vi "Write Scalar Data.vi"(8 "error in (no error)":errorcluster, 9 "Changed?":bool[](array[boolean]), 10 "Values":dbl[](array[numeric]), 11 "Cluster":T1 {"Data Type" format="%.0x"}) -> (0 "error out":errorcluster, 2 "Values":dbl[](array[numeric]), 3 "Cluster":T1 {"Data Type" format="%.0x"})   [LabVIEW 2019, in "FPGA Addon Engine.lvlib"]
uses:
  FPGA Addon Engine.lvlib
  Types/Register Settings.ctl
  Addon Shared/Types/Data Type.ctl
  Addon Shared/Types/Scalar Type.ctl
  <vilib>/Utility/error.llb/Error Cluster From Error Code.vi
  <vilib>/rvi/errors/niLvFpgaAdjustHostInterfaceError.vi
  <vilib>/rvi/interface/nirviReadWriteControl/nirviReadWriteControl.xnode
  <vilib>/rvi/interface/Simulation/niFpgaSimulationCallBeginRW.vi
  NiFpgaLv.dll
  Addon Shared/FPGA Addon Shared.lvlib
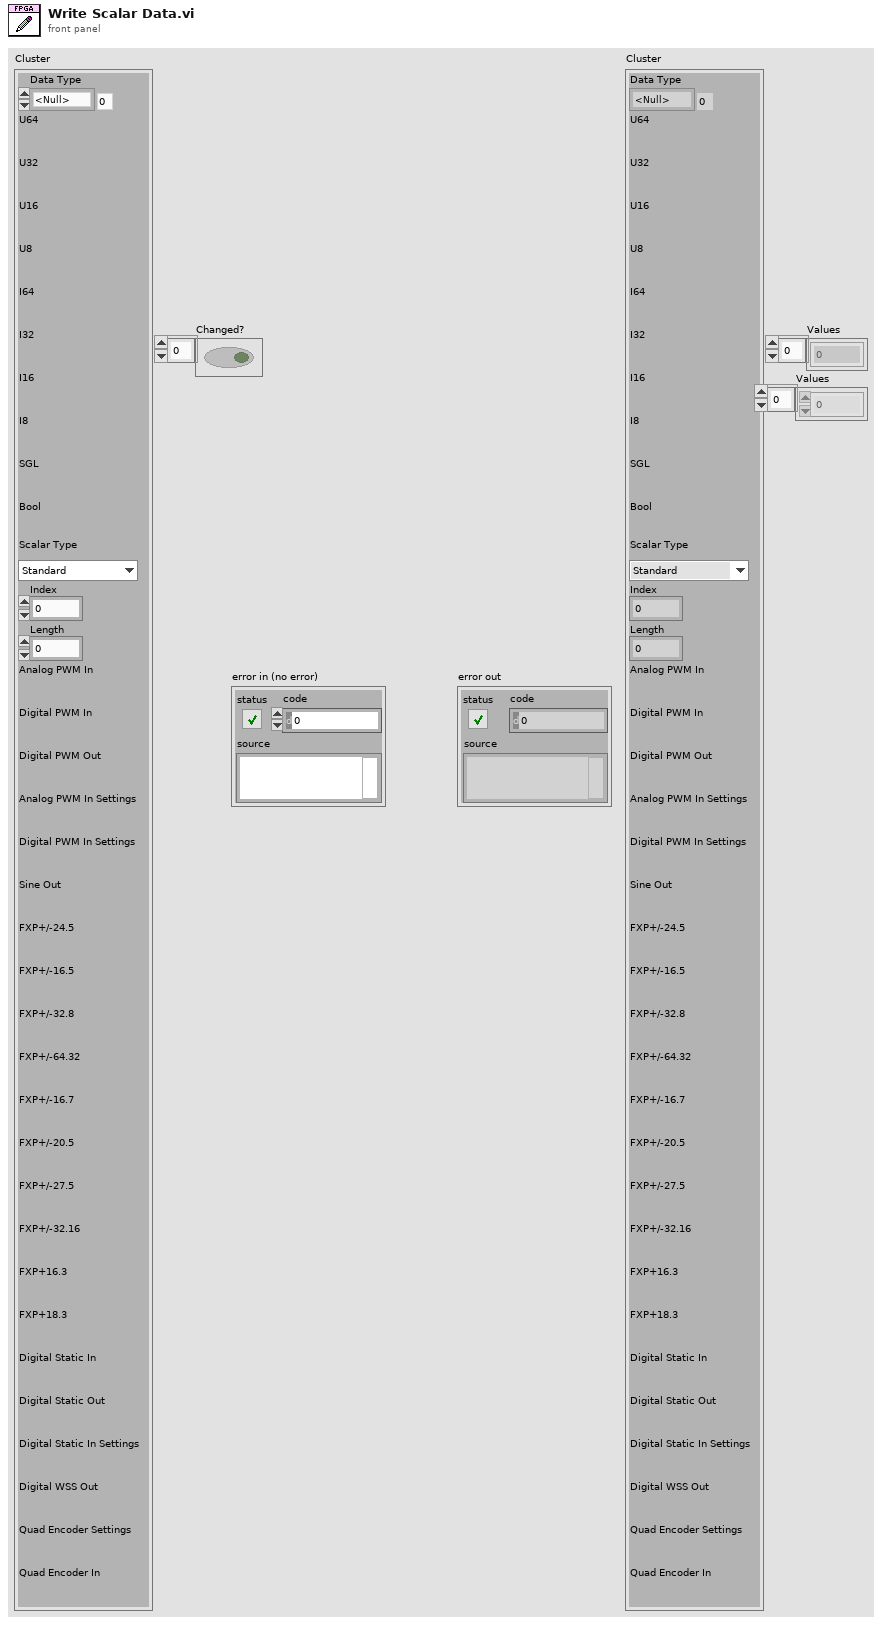
[diagram p1: front panel]
types:
  T1 = typedef "FPGA Addon Engine.lvlib/Register Settings.ctl" = cluster{"Data Type":T2, "U64":refnum<k20>, "U32":refnum<k20>, "U16":refnum<k20>, "U8":refnum<k20>, "I64":refnum<k20>, "I32":refnum<k20>, "I16":refnum<k20>, "I8":refnum<k20>, "SGL":refnum<k20>, "Bool":refnum<k20>, "Scalar Type":T3, "Index":i32, "Length":i32, "Analog PWM In":refnum<k20>, "Digital PWM In":refnum<k20>, "Digital PWM Out":refnum<k20>, "Analog PWM In Settings":refnum<k20>, "Digital PWM In Settings":refnum<k20>, "Sine Out":refnum<k20>, "FXP+/-24.5":refnum<k20>, "FXP+/-16.5":refnum<k20>, "FXP+/-32.8":refnum<k20>, "FXP+/-64.32":refnum<k20>, "FXP+/-16.7":refnum<k20>, "FXP+/-20.5":refnum<k20>, "FXP+/-27.5":refnum<k20>, "FXP+/-32.16":refnum<k20>, "FXP+16.3":refnum<k20>, "FXP+18.3":refnum<k20>, "Digital Static In":refnum<k20>, "Digital Static Out":refnum<k20>, "Digital Static In Settings":refnum<k20>, "Digital WSS Out":refnum<k20>, "Quad Encoder Settings":refnum<k20>, "Quad Encoder In":refnum<k20>}
  T2 = typedef "FPGA Addon Shared.lvlib/Data Type.ctl" = enum8{"<Null>", "I8", "I16", "I32", "I64", "U8", "U16", "U32", "U64", "SGL", "Boolean", "Analog PWM In Settings", "Analog PWM In", "Digital PWM In Settings", "Digital PWM In", "Digital PWM Out", "Sine Out", "FXP+/-24.5", "FXP+/-16.5", "FXP+/-32.8", "FXP+/-64.32", "FXP+/-16.7", "FXP+/-20.5", "FXP+/-27.5", "FXP+/-32.16", "FXP +16.3", "FXP +18.3", "Digital Static In", "Digital Static Out", "Digital Static In Settings", "Digital WSS Out", "Quad Encoder Settings", "Quad Encoder In"}
  T3 = typedef "FPGA Addon Shared.lvlib/Scalar Type.ctl" = enum16{"Standard", "Bitpacked"}
  T4 = cluster{"ACTIVE EDGE":bool, "TIMEOUT":u32, "THRESHOLD":fxp<+/-,32,8>}
  T5 = cluster{"ACTIVE EDGE":bool, "ACTIVE TICKS":u32, "INACTIVE TICKS":u32}
  T6 = cluster{"ACTIVE EDGE":bool, "ACTIVE TICKS":u32, "INACTIVE TICKS":u32, "DATA":u8, "SENSOR TYPE":u8}
  T7 = cluster{"AMP":fxp<+/-,32,8>, "OFFSET":fxp<+/-,32,8>, "PERIODS/TICKS":fxp<+,32,0>}
  T8 = cluster{"DIRECTION":u8, "RESET VALUE":i32, "A RESET STATE":bool, "B RESET STATE":bool, "Z RESET STATE":bool}
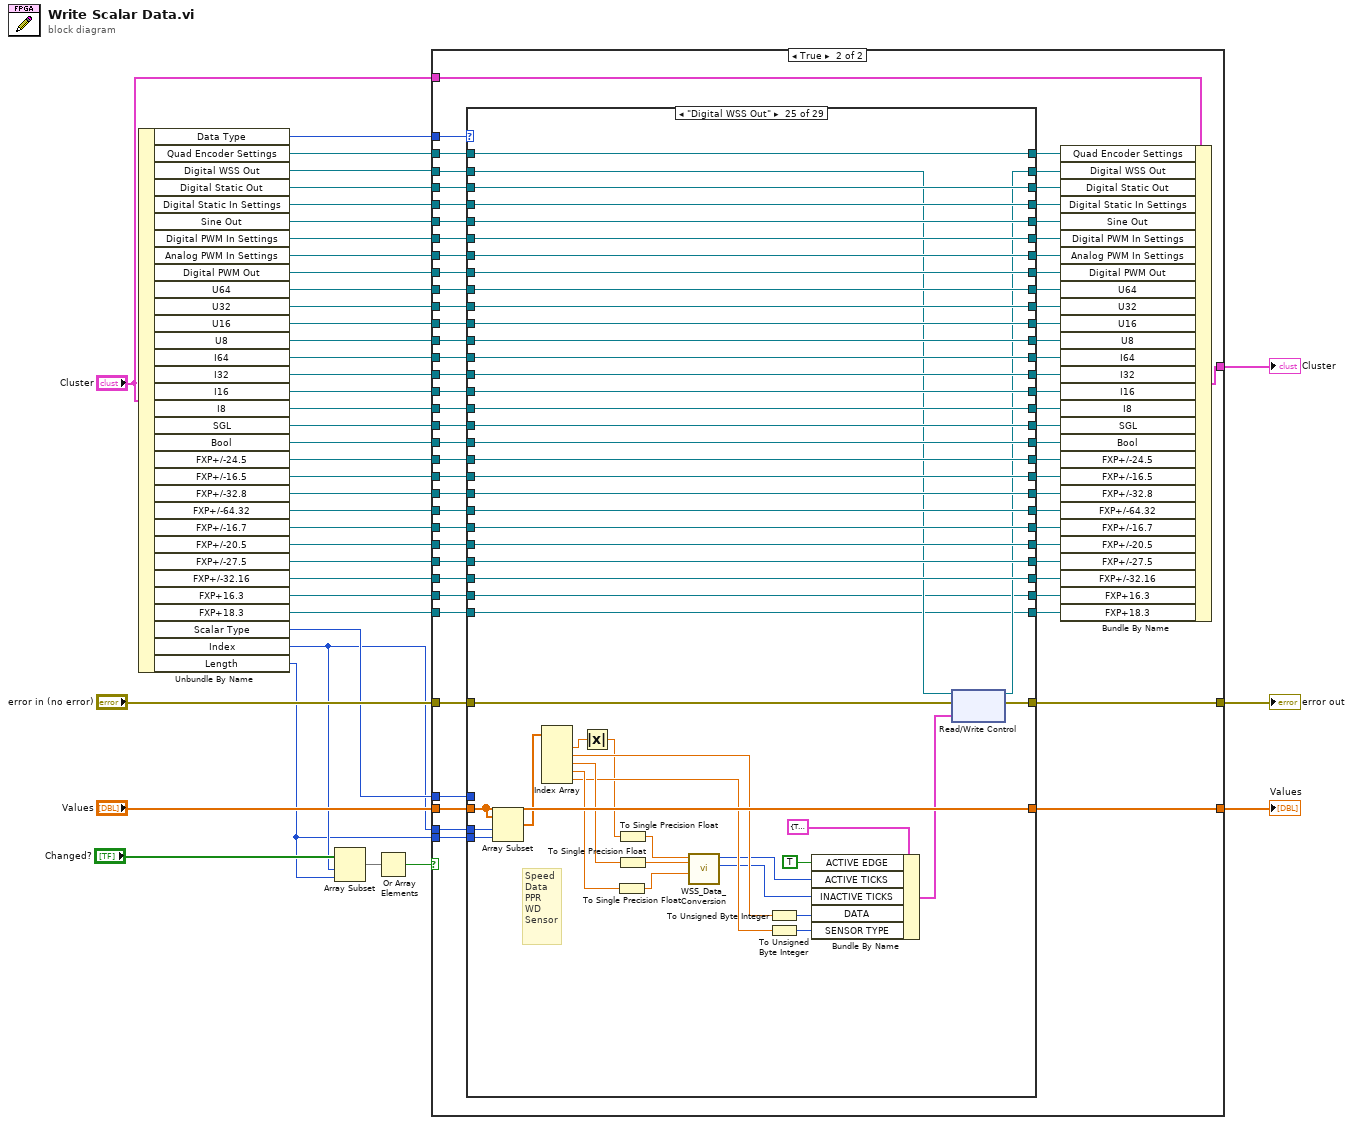
[diagram p0: block diagram]
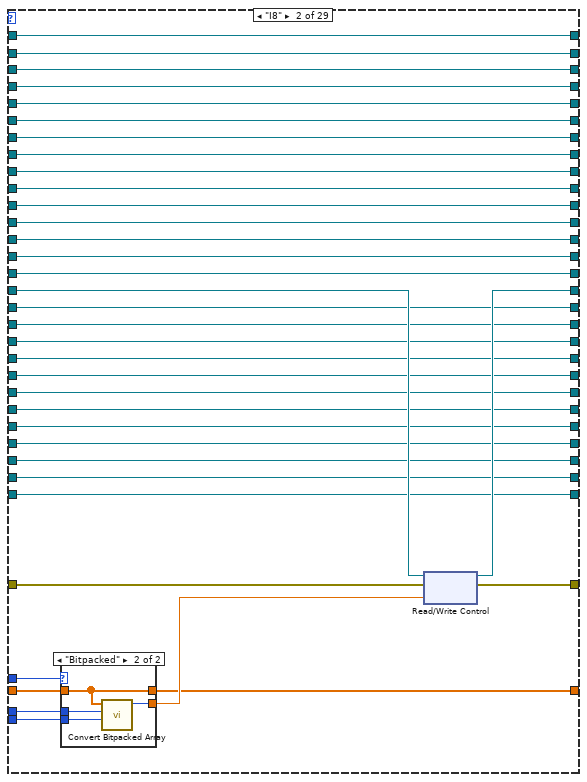
[diagram p4: hidden frame]
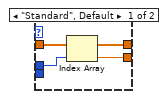
[diagram p5: hidden frame]
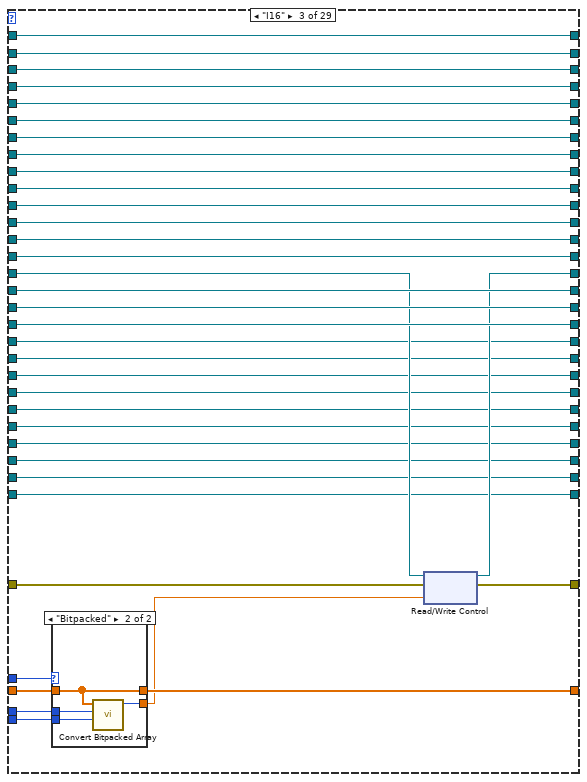
[diagram p6: hidden frame]
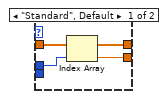
[diagram p7: hidden frame]
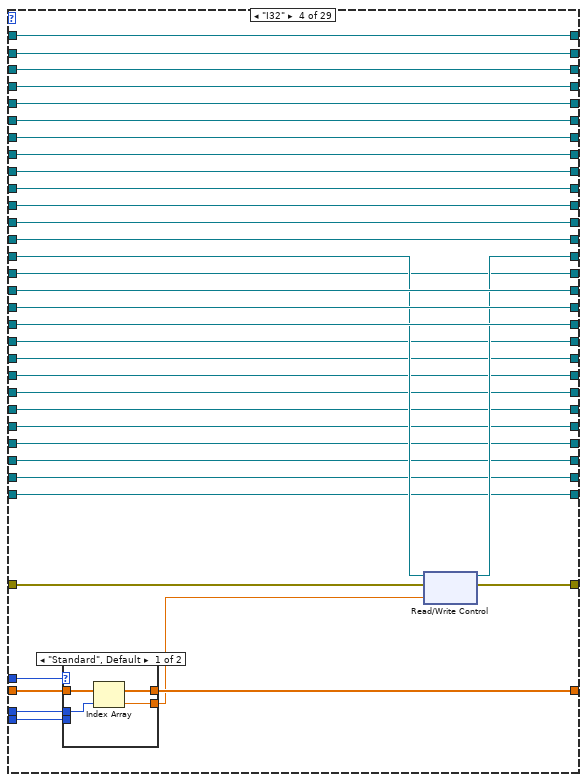
[diagram p8: hidden frame]
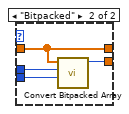
[diagram p9: hidden frame]
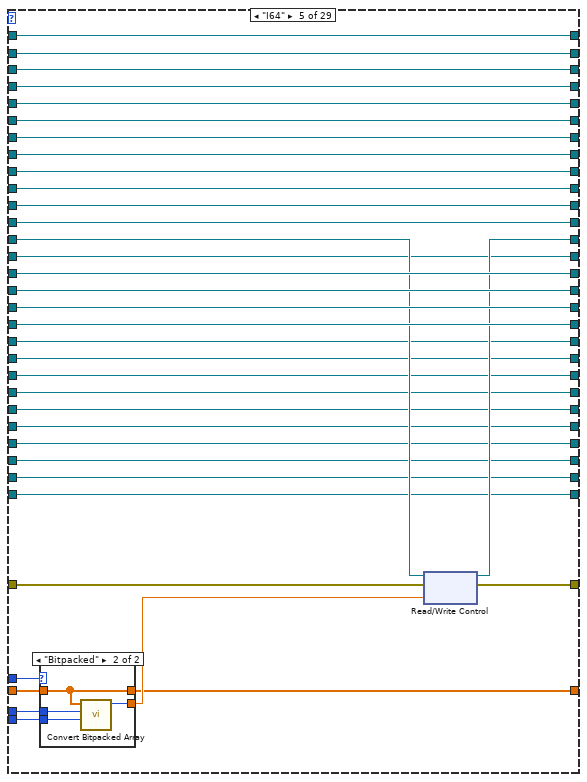
[diagram p10: hidden frame]
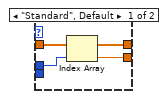
[diagram p11: hidden frame]
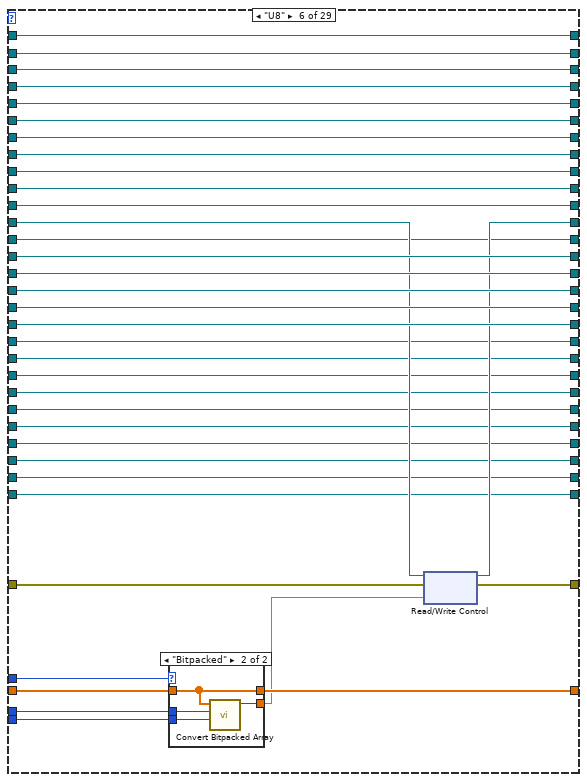
[diagram p12: hidden frame]
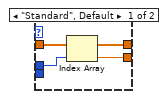
[diagram p13: hidden frame]
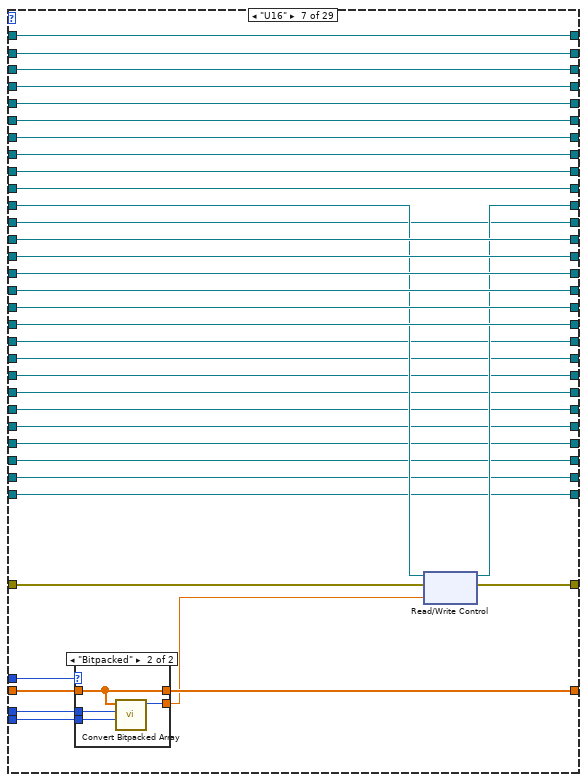
[diagram p14: hidden frame]
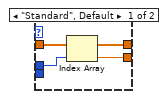
[diagram p15: hidden frame]
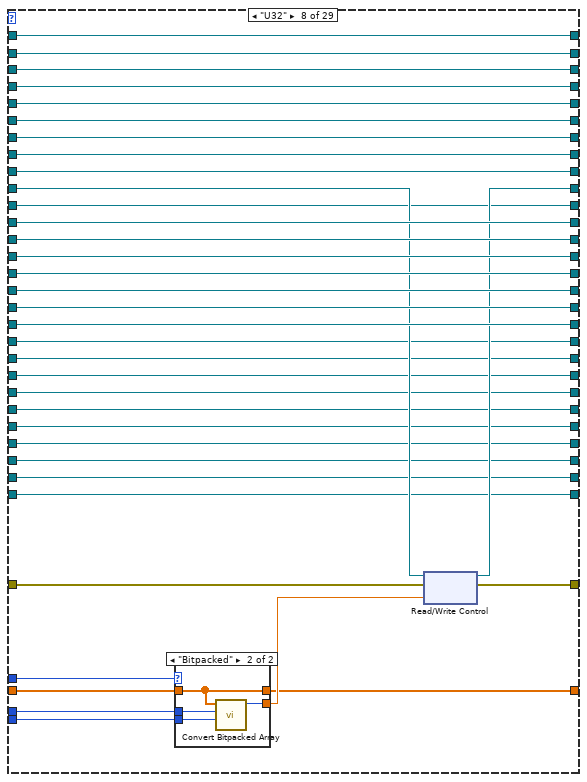
[diagram p16: hidden frame]
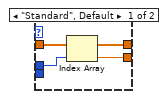
[diagram p17: hidden frame]
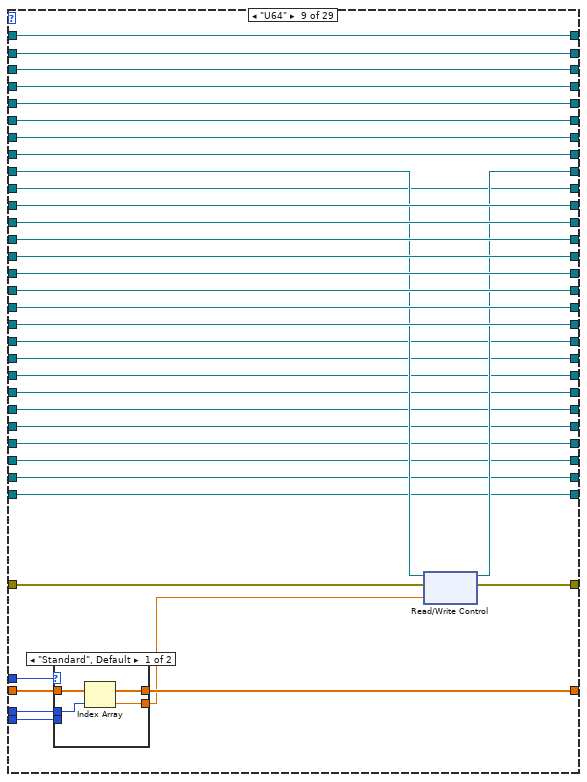
[diagram p18: hidden frame]
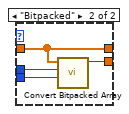
[diagram p19: hidden frame]
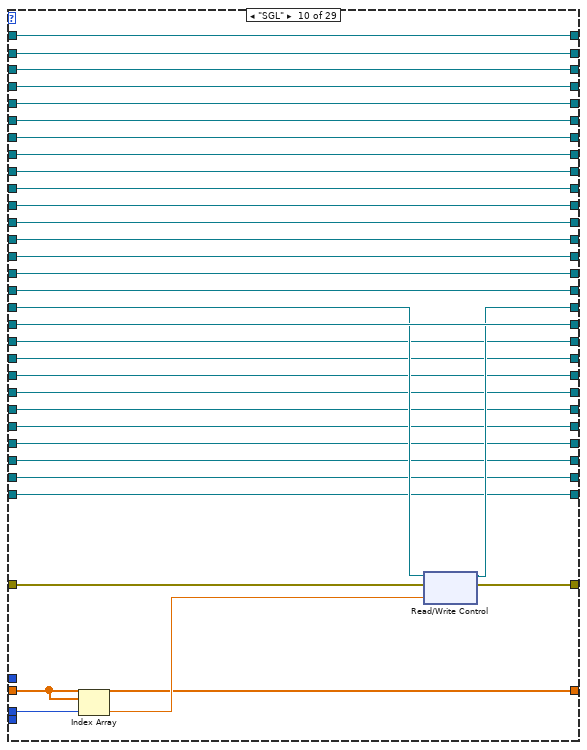
[diagram p20: hidden frame]
diagram:
  n1 = Unbundle By Name("Cluster") -> ("Data Type"=w4:T2, "Quad Encoder Settings"=w3:refnum<k20>, "Digital WSS Out"=w5:refnum<k20>, "Digital Static Out"=w7:refnum<k20>, "Digital Static In Settings"=w6:refnum<k20>, "Sine Out"=w16:refnum<k20>, "Digital PWM In Settings"=w22:refnum<k20>, "Analog PWM In Settings"=w23:refnum<k20>, "Digital PWM Out"=w24:refnum<k20>, "U64"=w29:refnum<k20>, "U32"=w30:refnum<k20>, "U16"=w31:refnum<k20>, "U8"=w32:refnum<k20>, "I64"=w33:refnum<k20>, "I32"=w34:refnum<k20>, "I16"=w35:refnum<k20>, "I8"=w41:refnum<k20>, "SGL"=w37:refnum<k20>, "Bool"=w36:refnum<k20>, "FXP+/-24.5"=w12:refnum<k20>, "FXP+/-16.5"=w13:refnum<k20>, "FXP+/-32.8"=w14:refnum<k20>, "FXP+/-64.32"=w15:refnum<k20>, "FXP+/-16.7"=w11:refnum<k20>, "FXP+/-20.5"=w10:refnum<k20>, "FXP+/-27.5"=w9:refnum<k20>, "FXP+/-32.16"=w8:refnum<k20>, "FXP+16.3"=w2:refnum<k20>, "FXP+18.3"=w1:refnum<k20>, "Scalar Type"=w25:T3, "Index"=w20:i32, "Length"=w19:i32)
  n2 = Array Subset(array="Changed?", index=w20, length=w19) -> (w18:bool[])
  n3 = Or Array Elements(Boolean array=w18) -> (logical OR=w17:bool)
  n4 = case shown="True" w17 {
    tunnel: w41 -> [_ w110]
    tunnel: "error in (no error)" -> [w43 w109]
    tunnel: [w43 w108] -> w39
    tunnel: "Cluster" -> [w44 w107]
    tunnel: w37 -> [_ w104]
    tunnel: w36 -> [_ w103]
    tunnel: w35 -> [_ w100]
    tunnel: w34 -> [_ w98]
    tunnel: w33 -> [_ w96]
    tunnel: w32 -> [_ w94]
    tunnel: w31 -> [_ w92]
    tunnel: w30 -> [_ w90]
    tunnel: w29 -> [_ w88]
    tunnel: [w44 w87] -> w28
    tunnel: [w42 w86] -> w27
    tunnel: "Values" -> [w42 w85]
    tunnel: w25 -> [_ w84]
    tunnel: w24 -> [_ w82]
    tunnel: w23 -> [_ w81]
    tunnel: w22 -> [_ w78]
    tunnel: w20 -> [_ w77]
    tunnel: w19 -> [_ w76]
    tunnel: w16 -> [_ w75]
    tunnel: w15 -> [_ w72]
    tunnel: w14 -> [_ w71]
    tunnel: w13 -> [_ w68]
    tunnel: w12 -> [_ w67]
    tunnel: w11 -> [_ w65]
    tunnel: w10 -> [_ w63]
    tunnel: w9 -> [_ w61]
    tunnel: w8 -> [_ w59]
    tunnel: w7 -> [_ w57]
    tunnel: w6 -> [_ w54]
    tunnel: w5 -> [_ w53]
    tunnel: w4 -> [_ w51]
    tunnel: w3 -> [_ w49]
    tunnel: w2 -> [_ w47]
    tunnel: w1 -> [_ w45]
    frame False {
    }
    frame True {
      n5 = case shown="\"Digital WSS Out\"" w51 {
        tunnel: w110 -> [w138 w177 w211 w256 w301 w346 w391 w436 w481 w523 w560 w594 w628 w662 w696 w730 w764 w798 w832 w866 w900 w935 w977 w1042 w1096 w1138 w1178 w1220 w1266]
        tunnel: w109 -> [w130 w176 w221 w265 w309 w353 w397 w441 w485 w526 w562 w596 w630 w664 w698 w732 w766 w800 w834 w868 w902 w932 w974 w1030 w1084 w1126 w1150 w1208 w1254]
        tunnel: [w130 w175 w220 w264 w308 w352 w396 w440 w484 w525 w561 w595 w629 w663 w697 w731 w765 w799 w833 w867 w901 w931 w973 w1029 w1083 w1125 w1151 w1207 w1253] -> w108
        tunnel: [w138 w174 w211 w256 w301 w346 w391 w436 w481 w523 w560 w594 w628 w662 w696 w730 w764 w798 w832 w866 w900 w935 w977 w1042 w1096 w1138 w1178 w1220 w1266] -> w106
        tunnel: [w139 w173 w219 w263 w307 w351 w395 w439 w483 w514 w550 w586 w620 w654 w688 w722 w756 w790 w824 w858 w892 w934 w976 w1041 w1095 w1137 w1177 w1219 w1265] -> w105
        tunnel: w104 -> [w139 w173 w219 w263 w307 w351 w395 w439 w483 w516 w550 w586 w620 w654 w688 w722 w756 w790 w824 w858 w892 w934 w976 w1041 w1095 w1137 w1177 w1219 w1265]
        tunnel: w103 -> [w140 w172 w218 w262 w306 w350 w394 w438 w482 w524 w552 w575 w610 w645 w680 w714 w749 w783 w817 w851 w885 w933 w975 w1040 w1094 w1136 w1176 w1218 w1264]
        tunnel: [w140 w172 w218 w262 w306 w350 w394 w438 w482 w524 w551 w575 w610 w645 w680 w714 w749 w783 w817 w851 w885 w933 w975 w1040 w1094 w1136 w1176 w1218 w1264] -> w102
        tunnel: [w137 w171 w209 w253 w300 w345 w390 w435 w480 w522 w559 w593 w627 w661 w695 w729 w763 w797 w831 w865 w899 w936 w978 w1039 w1093 w1135 w1175 w1217 w1263] -> w101
        tunnel: w100 -> [w137 w171 w210 w253 w300 w345 w390 w435 w480 w522 w559 w593 w627 w661 w695 w729 w763 w797 w831 w865 w899 w936 w978 w1039 w1093 w1135 w1175 w1217 w1263]
        tunnel: [w136 w170 w217 w254 w297 w344 w389 w434 w479 w521 w558 w592 w626 w660 w694 w728 w762 w796 w830 w864 w898 w937 w979 w1038 w1092 w1134 w1174 w1216 w1262] -> w99
        tunnel: w98 -> [w136 w170 w217 w255 w297 w344 w389 w434 w479 w521 w558 w592 w626 w660 w694 w728 w762 w796 w830 w864 w898 w937 w979 w1038 w1092 w1134 w1174 w1216 w1262]
        tunnel: [w135 w169 w216 w261 w298 w341 w388 w433 w478 w520 w557 w591 w625 w659 w693 w727 w761 w795 w829 w863 w897 w938 w980 w1037 w1091 w1133 w1173 w1215 w1261] -> w97
        tunnel: w96 -> [w135 w169 w216 w261 w299 w341 w388 w433 w478 w520 w557 w591 w625 w659 w693 w727 w761 w795 w829 w863 w897 w938 w980 w1037 w1091 w1133 w1173 w1215 w1261]
        tunnel: [w134 w168 w215 w260 w305 w342 w385 w432 w477 w519 w556 w590 w624 w658 w692 w726 w760 w794 w828 w862 w896 w939 w981 w1036 w1090 w1132 w1172 w1214 w1260] -> w95
        tunnel: w94 -> [w134 w168 w215 w260 w305 w343 w385 w432 w477 w519 w556 w590 w624 w658 w692 w726 w760 w794 w828 w862 w896 w939 w981 w1036 w1090 w1132 w1172 w1214 w1260]
        tunnel: [w133 w167 w214 w259 w304 w349 w386 w429 w476 w518 w555 w589 w623 w657 w691 w725 w759 w793 w827 w861 w895 w940 w982 w1035 w1089 w1131 w1171 w1213 w1259] -> w93
        tunnel: w92 -> [w133 w167 w214 w259 w304 w349 w387 w429 w476 w518 w555 w589 w623 w657 w691 w725 w759 w793 w827 w861 w895 w940 w982 w1035 w1089 w1131 w1171 w1213 w1259]
        tunnel: [w132 w166 w213 w258 w303 w348 w393 w430 w473 w517 w554 w588 w622 w656 w690 w724 w758 w792 w826 w860 w894 w941 w983 w1034 w1088 w1130 w1170 w1212 w1258] -> w91
        tunnel: w90 -> [w132 w166 w213 w258 w303 w348 w393 w431 w473 w517 w554 w588 w622 w656 w690 w724 w758 w792 w826 w860 w894 w941 w983 w1034 w1088 w1130 w1170 w1212 w1258]
        tunnel: [w131 w165 w212 w257 w302 w347 w392 w437 w474 w515 w553 w587 w621 w655 w689 w723 w757 w791 w825 w859 w893 w942 w984 w1033 w1087 w1129 w1169 w1211 w1257] -> w89
        tunnel: w88 -> [w131 w165 w212 w257 w302 w347 w392 w437 w475 w515 w553 w587 w621 w655 w689 w723 w757 w791 w825 w859 w893 w942 w984 w1033 w1087 w1129 w1169 w1211 w1257]
        tunnel: [w129 w159 w204 w248 w291 w336 w380 w423 w468 w511 w547 w585 w619 w653 w687 w721 w755 w789 w823 w857 w891 w926 w970 w1023 w1082 w1124 w1166 w1206 w1252] -> w86
        tunnel: w85 -> [w129 w164 w208 w252 w296 w340 w384 w428 w472 w511 w547 w585 w619 w653 w687 w721 w755 w789 w823 w857 w891 w926 w970 w1023 w1082 w1124 w1166 w1206 w1252]
        tunnel: w76 -> [_ w162 w206 w249 w293 w339 w382 w426 w469 _ _ _ _ _ _ _ _ _ _ _ _ w927 w971 w1022 w1081 w1123 w1165 w1205 w1251]
        tunnel: w84 -> [_ w161 w205 w251 w295 w337 w381 w425 w471 _ _ _ _ _ _ _ _ _ _ _ _ _ _ _ _ _ _ _ _]
        tunnel: w77 -> [_ w163 w207 w250 w294 w338 w383 w427 w470 w513 w546 w584 w618 w652 w686 w720 w754 w788 w822 w856 w890 w928 w972 w1021 w1080 w1122 w1164 w1204 w1250]
        tunnel: [w128 w156 w200 w244 w288 w332 w376 w420 w464 w508 w542 w581 w615 w649 w683 w717 w751 w785 w819 w853 w887 w944 w985 w1027 w1066 w1118 w1163 w1202 w1248] -> w83
        tunnel: w82 -> [w128 w156 w200 w244 w288 w332 w376 w420 w464 w508 w542 w581 w615 w649 w683 w717 w751 w785 w819 w853 w887 w944 w985 w1028 w1066 w1118 w1163 w1202 w1248]
        tunnel: w81 -> [w127 w157 w201 w245 w289 w333 w377 w421 w465 w509 w543 w582 w616 w650 w684 w718 w752 w786 w820 w854 w888 w930 w964 w1032 w1086 w1128 w1168 w1210 w1256]
        tunnel: [w127 w157 w201 w245 w289 w333 w377 w421 w465 w509 w543 w582 w616 w650 w684 w718 w752 w786 w820 w854 w888 w929 w964 w1032 w1086 w1128 w1168 w1210 w1256] -> w80
        tunnel: [w126 w158 w202 w246 w290 w334 w378 w422 w466 w510 w544 w583 w617 w651 w685 w719 w753 w787 w821 w855 w889 w943 w966 w1031 w1085 w1127 w1167 w1209 w1255] -> w79
        tunnel: w78 -> [w126 w158 w202 w246 w290 w334 w378 w422 w466 w510 w544 w583 w617 w651 w685 w719 w753 w787 w821 w855 w889 w943 w965 w1031 w1085 w1127 w1167 w1209 w1255]
        tunnel: w75 -> [w125 w155 w199 w243 w287 w331 w375 w419 w463 w507 w541 w580 w614 w648 w682 w716 w750 w784 w818 w852 w886 w919 w961 w1002 w1078 w1120 w1148 w1193 w1239]
        tunnel: [w125 w155 w199 w243 w287 w331 w375 w419 w463 w507 w541 w580 w614 w648 w682 w716 w750 w784 w818 w852 w886 w919 w961 w1002 w1078 w1119 w1148 w1193 w1239] -> w74
        tunnel: [w124 w154 w198 w242 w286 w330 w374 w418 w462 w506 w540 w579 w613 w647 w675 w710 w745 w779 w813 w847 w881 w918 w958 w999 w1076 w1110 w1162 w1201 w1247] -> w73
        tunnel: w72 -> [w124 w154 w198 w242 w286 w330 w374 w418 w462 w506 w540 w579 w613 w647 w677 w710 w745 w779 w813 w847 w881 w918 w958 w999 w1076 w1110 w1162 w1201 w1247]
        tunnel: w71 -> [w123 w153 w197 w241 w285 w329 w373 w417 w461 w505 w539 w578 w612 w641 w676 w711 w746 w780 w814 w848 w882 w917 w957 w998 w1075 w1109 w1161 w1200 w1246]
        tunnel: [w123 w153 w197 w241 w285 w329 w373 w417 w461 w505 w539 w578 w612 w642 w676 w711 w746 w780 w814 w848 w882 w917 w957 w998 w1075 w1109 w1161 w1200 w1246] -> w70
        tunnel: [w122 w152 w196 w240 w284 w328 w372 w416 w460 w504 w538 w577 w607 w643 w678 w712 w747 w781 w815 w849 w883 w916 w956 w997 w1074 w1108 w1160 w1199 w1245] -> w69
        tunnel: w68 -> [w122 w152 w196 w240 w284 w328 w372 w416 w460 w504 w538 w577 w608 w643 w678 w712 w747 w781 w815 w849 w883 w916 w956 w997 w1074 w1108 w1160 w1199 w1245]
        tunnel: w67 -> [w121 w151 w195 w239 w283 w327 w371 w415 w459 w503 w537 w574 w609 w644 w679 w713 w748 w782 w816 w850 w884 w915 w955 w996 w1073 w1107 w1159 w1198 w1244]
        tunnel: [w121 w151 w195 w239 w283 w327 w371 w415 w459 w503 w537 w573 w609 w644 w679 w713 w748 w782 w816 w850 w884 w915 w955 w996 w1073 w1107 w1159 w1198 w1244] -> w66
        tunnel: w65 -> [w120 w150 w194 w238 w282 w326 w370 w414 w458 w502 w536 w572 w606 w640 w674 w709 w743 w778 w812 w846 w880 w914 w954 w995 w1072 w1106 w1158 w1197 w1243]
        tunnel: [w120 w150 w194 w238 w282 w326 w370 w414 w458 w502 w536 w572 w606 w640 w674 w708 w743 w778 w812 w846 w880 w914 w954 w995 w1072 w1106 w1158 w1197 w1243] -> w64
        tunnel: w63 -> [w119 w149 w193 w237 w281 w325 w369 w413 w457 w501 w535 w571 w605 w639 w673 w707 w744 w775 w810 w844 w878 w911 w953 w994 w1071 w1105 w1157 w1196 w1242]
        tunnel: [w119 w149 w193 w237 w281 w325 w369 w413 w457 w501 w535 w571 w605 w639 w673 w707 w742 w775 w810 w844 w878 w911 w953 w994 w1071 w1105 w1157 w1196 w1242] -> w62
        tunnel: w61 -> [w118 w148 w192 w236 w280 w324 w368 w412 w456 w500 w534 w570 w604 w638 w672 w706 w740 w776 w807 w843 w877 w910 w952 w993 w1070 w1104 w1156 w1195 w1241]
        tunnel: [w118 w148 w192 w236 w280 w324 w368 w412 w456 w500 w534 w570 w604 w638 w672 w706 w740 w774 w807 w843 w877 w910 w952 w993 w1070 w1104 w1156 w1195 w1241] -> w60
        tunnel: w59 -> [w117 w147 w191 w235 w279 w323 w367 w411 w455 w499 w533 w569 w603 w637 w671 w705 w739 w773 w809 w838 w872 w909 w951 w992 w1069 w1103 w1155 w1194 w1240]
        tunnel: [w117 w147 w191 w235 w279 w323 w367 w411 w455 w499 w533 w569 w603 w637 w671 w705 w739 w773 w808 w838 w872 w909 w951 w992 w1069 w1103 w1155 w1194 w1240] -> w58
        tunnel: w57 -> [w116 w146 w190 w234 w278 w322 w366 w410 w454 w498 w532 w568 w602 w636 w670 w704 w738 w772 w806 w842 w876 w908 w950 w991 w1068 w1102 w1143 w1191 w1233]
        tunnel: [w116 w146 w190 w234 w278 w322 w366 w410 w454 w498 w532 w568 w602 w636 w670 w704 w738 w772 w806 w842 w876 w908 w950 w991 w1068 w1102 w1143 w1190 w1233] -> w56
        tunnel: [w115 w145 w189 w233 w277 w321 w365 w409 w453 w497 w531 w567 w601 w635 w669 w703 w737 w771 w805 w841 w875 w907 w949 w990 w1067 w1101 w1144 w1192 w1238] -> w55
        tunnel: w54 -> [w115 w145 w189 w233 w277 w321 w365 w409 w453 w497 w531 w567 w601 w635 w669 w703 w737 w771 w805 w841 w875 w907 w949 w990 w1067 w1101 w1147 w1192 w1238]
        tunnel: w53 -> [w114 w144 w188 w232 w276 w320 w364 w408 w452 w496 w530 w566 w600 w634 w668 w702 w736 w770 w804 w840 w874 w906 w948 w989 w1064 w1100 w1142 w1182 w1235]
        tunnel: [w114 w144 w188 w232 w276 w320 w364 w408 w452 w496 w530 w566 w600 w634 w668 w702 w736 w770 w804 w840 w874 w906 w948 w989 w1065 w1100 w1142 w1182 w1235] -> w52
        tunnel: [w113 w143 w187 w231 w275 w319 w363 w407 w451 w495 w529 w565 w599 w633 w667 w701 w735 w769 w803 w839 w873 w905 w947 w988 w1049 w1099 w1141 w1181 w1232] -> w50
        tunnel: w49 -> [w113 w143 w187 w231 w275 w319 w363 w407 w451 w495 w529 w565 w599 w633 w667 w701 w735 w769 w803 w839 w873 w905 w947 w988 w1049 w1099 w1141 w1181 w1234]
        tunnel: [w112 w142 w186 w230 w274 w318 w362 w406 w450 w494 w528 w564 w598 w632 w666 w700 w734 w768 w802 w836 w871 w904 w946 w987 w1048 w1098 w1140 w1180 w1222] -> w48
        tunnel: w47 -> [w112 w142 w186 w230 w274 w318 w362 w406 w450 w494 w528 w564 w598 w632 w666 w700 w734 w768 w802 w837 w871 w904 w946 w987 w1048 w1098 w1140 w1180 w1222]
        tunnel: [w111 w141 w185 w229 w273 w317 w361 w405 w449 w493 w527 w563 w597 w631 w665 w699 w733 w767 w801 w835 w869 w903 w945 w986 w1047 w1097 w1139 w1179 w1221] -> w46
        tunnel: w45 -> [w111 w141 w185 w229 w273 w317 w361 w405 w449 w493 w527 w563 w597 w631 w665 w699 w733 w767 w801 w835 w870 w903 w945 w986 w1047 w1097 w1139 w1179 w1221]
        frame "<Null>", Default {
        }
        frame "I8" {
          n6 = case shown="\"Bitpacked\"" w161 {
            tunnel: w164 -> [w178 w181]
            tunnel: w163 -> [w180 w184]
            tunnel: [w179 w182] -> w160
            tunnel: w162 -> [_ w183]
            tunnel: [w178 w181] -> w159
            frame "Standard", Default {
              n7 = Index Array(array=w178, index=w180) -> (element=w179:dbl)
            }
            frame "Bitpacked" {
              n8 = call "Convert Bitpacked Array.vi"("Length"=w183, "Index"=w184, "Values"=w181) -> ("Numeric"=w182:u64)  [unwired: 8 in]
            }
          }
          n9 = xnode "Read/Write Control"("FPGA VI Reference In"=w177, "error in"=w176, "Value"=w160) -> ("FPGA VI Reference Out"=w174:refnum<k20>, "error out"=w175:errorcluster)
        }
        frame "I16" {
          n10 = case shown="\"Bitpacked\"" w205 {
            tunnel: w208 -> [w222 w225]
            tunnel: w207 -> [w224 w228]
            tunnel: [w223 w226] -> w203
            tunnel: w206 -> [_ w227]
            tunnel: [w222 w225] -> w204
            frame "Standard", Default {
              n11 = Index Array(array=w222, index=w224) -> (element=w223:dbl)
            }
            frame "Bitpacked" {
              n12 = call "Convert Bitpacked Array.vi"("Length"=w227, "Index"=w228, "Values"=w225) -> ("Numeric"=w226:u64)  [unwired: 8 in]
            }
          }
          n13 = xnode "Read/Write Control"("FPGA VI Reference In"=w210, "error in"=w221, "Value"=w203) -> ("FPGA VI Reference Out"=w209:refnum<k20>, "error out"=w220:errorcluster)
        }
        frame "I32" {
          n14 = case shown="\"Standard\", Default" w251 {
            tunnel: w252 -> [w266 w269]
            tunnel: w250 -> [w268 w272]
            tunnel: [w267 w270] -> w247
            tunnel: w249 -> [_ w271]
            tunnel: [w266 w269] -> w248
            frame "Standard", Default {
              n15 = Index Array(array=w266, index=w268) -> (element=w267:dbl)
            }
            frame "Bitpacked" {
              n16 = call "Convert Bitpacked Array.vi"("Length"=w271, "Index"=w272, "Values"=w269) -> ("Numeric"=w270:u64)  [unwired: 8 in]
            }
          }
          n17 = xnode "Read/Write Control"("FPGA VI Reference In"=w255, "error in"=w265, "Value"=w247) -> ("FPGA VI Reference Out"=w254:refnum<k20>, "error out"=w264:errorcluster)
        }
        frame "I64" {
          n18 = case shown="\"Bitpacked\"" w295 {
            tunnel: w296 -> [w310 w313]
            tunnel: w294 -> [w312 w316]
            tunnel: [w311 w314] -> w292
            tunnel: w293 -> [_ w315]
            tunnel: [w310 w313] -> w291
            frame "Standard", Default {
              n19 = Index Array(array=w310, index=w312) -> (element=w311:dbl)
            }
            frame "Bitpacked" {
              n20 = call "Convert Bitpacked Array.vi"("Length"=w315, "Index"=w316, "Values"=w313) -> ("Numeric"=w314:u64)  [unwired: 8 in]
            }
          }
          n21 = xnode "Read/Write Control"("FPGA VI Reference In"=w299, "error in"=w309, "Value"=w292) -> ("FPGA VI Reference Out"=w298:refnum<k20>, "error out"=w308:errorcluster)
        }
        frame "U8" {
          n22 = case shown="\"Bitpacked\"" w337 {
            tunnel: w340 -> [w354 w357]
            tunnel: w338 -> [w356 w360]
            tunnel: [w355 w358] -> w335
            tunnel: w339 -> [_ w359]
            tunnel: [w354 w357] -> w336
            frame "Standard", Default {
              n23 = Index Array(array=w354, index=w356) -> (element=w355:dbl)
            }
            frame "Bitpacked" {
              n24 = call "Convert Bitpacked Array.vi"("Length"=w359, "Index"=w360, "Values"=w357) -> ("Numeric"=w358:u64)  [unwired: 8 in]
            }
          }
          n25 = xnode "Read/Write Control"("FPGA VI Reference In"=w343, "error in"=w353, "Value"=w335) -> ("FPGA VI Reference Out"=w342:refnum<k20>, "error out"=w352:errorcluster)
        }
        frame "U16" {
          n26 = case shown="\"Bitpacked\"" w381 {
            tunnel: w384 -> [w398 w401]
            tunnel: w383 -> [w400 w404]
            tunnel: [w399 w402] -> w379
            tunnel: w382 -> [_ w403]
            tunnel: [w398 w401] -> w380
            frame "Standard", Default {
              n27 = Index Array(array=w398, index=w400) -> (element=w399:dbl)
            }
            frame "Bitpacked" {
              n28 = call "Convert Bitpacked Array.vi"("Length"=w403, "Index"=w404, "Values"=w401) -> ("Numeric"=w402:u64)  [unwired: 8 in]
            }
          }
          n29 = xnode "Read/Write Control"("FPGA VI Reference In"=w387, "error in"=w397, "Value"=w379) -> ("FPGA VI Reference Out"=w386:refnum<k20>, "error out"=w396:errorcluster)
        }
        frame "U32" {
          n30 = case shown="\"Bitpacked\"" w425 {
            tunnel: w428 -> [w442 w445]
            tunnel: w427 -> [w444 w448]
            tunnel: [w443 w446] -> w424
            tunnel: w426 -> [_ w447]
            tunnel: [w442 w445] -> w423
            frame "Standard", Default {
              n31 = Index Array(array=w442, index=w444) -> (element=w443:dbl)
            }
            frame "Bitpacked" {
              n32 = call "Convert Bitpacked Array.vi"("Length"=w447, "Index"=w448, "Values"=w445) -> ("Numeric"=w446:u64)  [unwired: 8 in]
            }
          }
          n33 = xnode "Read/Write Control"("FPGA VI Reference In"=w431, "error in"=w441, "Value"=w424) -> ("FPGA VI Reference Out"=w430:refnum<k20>, "error out"=w440:errorcluster)
        }
        frame "U64" {
          n34 = case shown="\"Standard\", Default" w471 {
            tunnel: w472 -> [w486 w489]
            tunnel: w470 -> [w488 w492]
            tunnel: [w487 w490] -> w467
            tunnel: w469 -> [_ w491]
            tunnel: [w486 w489] -> w468
            frame "Standard", Default {
              n35 = Index Array(array=w486, index=w488) -> (element=w487:dbl)
            }
            frame "Bitpacked" {
              n36 = call "Convert Bitpacked Array.vi"("Length"=w491, "Index"=w492, "Values"=w489) -> ("Numeric"=w490:u64)  [unwired: 8 in]
            }
          }
          n37 = xnode "Read/Write Control"("FPGA VI Reference In"=w475, "error in"=w485, "Value"=w467) -> ("FPGA VI Reference Out"=w474:refnum<k20>, "error out"=w484:errorcluster)
        }
        frame "SGL" {
          n38 = Index Array(array=w511, index=w513) -> (element=w512:dbl)
          n39 = xnode "Read/Write Control"("FPGA VI Reference In"=w516, "error in"=w526, "Value"=w512) -> ("FPGA VI Reference Out"=w514:refnum<k20>, "error out"=w525:errorcluster)
        }
        frame "Boolean" {
          n40 = Index Array(array=w547, index=w546) -> (element=w545:dbl)
          n41 = To Unsigned Byte Integer(number=w545) -> (unsigned 8bit integer=w548:u8)
          n42 = Greater Than 0?(x=w548) -> (x > 0?=w549:bool)
          n43 = xnode "Read/Write Control"("FPGA VI Reference In"=w552, "error in"=w562, "Value"=w549) -> ("FPGA VI Reference Out"=w551:refnum<k20>, "error out"=w561:errorcluster)
        }
        frame "FXP+/-24.5" {
          n44 = Index Array(array=w585, index=w584) -> (element=w576:dbl)
          n45 = xnode "Read/Write Control"("FPGA VI Reference In"=w574, "error in"=w596, "Value"=w576) -> ("FPGA VI Reference Out"=w573:refnum<k20>, "error out"=w595:errorcluster)
        }
        frame "FXP+/-16.5" {
          n46 = Index Array(array=w619, index=w618) -> (element=w611:dbl)
          n47 = xnode "Read/Write Control"("FPGA VI Reference In"=w608, "error in"=w630, "Value"=w611) -> ("FPGA VI Reference Out"=w607:refnum<k20>, "error out"=w629:errorcluster)
        }
        frame "FXP+/-32.8" {
          n48 = Index Array(array=w653, index=w652) -> (element=w646:dbl)
          n49 = xnode "Read/Write Control"("FPGA VI Reference In"=w641, "error in"=w664, "Value"=w646) -> ("FPGA VI Reference Out"=w642:refnum<k20>, "error out"=w663:errorcluster)
        }
        frame "FXP+/-64.32" {
          n50 = Index Array(array=w687, index=w686) -> (element=w681:dbl)
          n51 = xnode "Read/Write Control"("FPGA VI Reference In"=w677, "error in"=w698, "Value"=w681) -> ("FPGA VI Reference Out"=w675:refnum<k20>, "error out"=w697:errorcluster)
        }
        frame "FXP+/-16.7" {
          n52 = Index Array(array=w721, index=w720) -> (element=w715:dbl)
          n53 = xnode "Read/Write Control"("FPGA VI Reference In"=w709, "error in"=w732, "Value"=w715) -> ("FPGA VI Reference Out"=w708:refnum<k20>, "error out"=w731:errorcluster)
        }
        frame "FXP+/-20.5" {
          n54 = Index Array(array=w755, index=w754) -> (element=w741:dbl)
          n55 = xnode "Read/Write Control"("FPGA VI Reference In"=w744, "error in"=w766, "Value"=w741) -> ("FPGA VI Reference Out"=w742:refnum<k20>, "error out"=w765:errorcluster)
        }
        frame "FXP+/-27.5" {
          n56 = Index Array(array=w789, index=w788) -> (element=w777:dbl)
          n57 = xnode "Read/Write Control"("FPGA VI Reference In"=w776, "error in"=w800, "Value"=w777) -> ("FPGA VI Reference Out"=w774:refnum<k20>, "error out"=w799:errorcluster)
        }
        frame "FXP+/-32.16" {
          n58 = Index Array(array=w823, index=w822) -> (element=w811:dbl)
          n59 = xnode "Read/Write Control"("FPGA VI Reference In"=w809, "error in"=w834, "Value"=w811) -> ("FPGA VI Reference Out"=w808:refnum<k20>, "error out"=w833:errorcluster)
        }
        frame "FXP +16.3" {
          n60 = Index Array(array=w857, index=w856) -> (element=w845:dbl)
          n61 = xnode "Read/Write Control"("FPGA VI Reference In"=w837, "error in"=w868, "Value"=w845) -> ("FPGA VI Reference Out"=w836:refnum<k20>, "error out"=w867:errorcluster)
        }
        frame "FXP +18.3" {
          n62 = Index Array(array=w891, index=w890) -> (element=w879:dbl)
          n63 = xnode "Read/Write Control"("FPGA VI Reference In"=w870, "error in"=w902, "Value"=w879) -> ("FPGA VI Reference Out"=w869:refnum<k20>, "error out"=w901:errorcluster)
        }
        frame "Analog PWM In Settings" {
          n64 = Array Subset(array=w926, index=w928, length=w927) -> (w925:dbl[])
          n65 = Index Array(array=w925) -> (element #1=w923:dbl, element #2=w921:dbl, element #3=w920:dbl)  [unwired: 4 in, 1 out]
          n66 = Greater?(x=w923, y=0.5) -> (0:w922:bool)
          n67 = Bundle By Name(cluster=T4 {"ACTIVE EDGE"=FALSE, "TIMEOUT"=0, "THRESHOLD"=0.0} ("Value"), "ACTIVE EDGE"=w922, "TIMEOUT"=w921, "THRESHOLD"=w920) -> (w912:T4)
          n68 = xnode "Read/Write Control"("FPGA VI Reference In"=w930, "error in"=w932, "Value"=w912) -> ("FPGA VI Reference Out"=w929:refnum<k20>, "error out"=w931:errorcluster)
        }
        frame "Digital PWM In Settings" {
          n69 = Array Subset(array=w970, index=w972, length=w971) -> (w969:dbl[])
          n70 = Index Array(array=w969) -> (element #1=w963:dbl, element #2=w962:dbl)  [unwired: 2 in]
          n71 = Greater?(x=w963, y=0.5) -> (0:w968:bool)
          n72 = Bundle By Name(cluster=cluster{"ACTIVE EDGE":bool, "TIMEOUT":u32} {"ACTIVE EDGE"=FALSE, "TIMEOUT"=0} ("Value"), "ACTIVE EDGE"=w968, "TIMEOUT"=w962) -> (w959:cluster{"ACTIVE EDGE":bool, "TIMEOUT":u32})
          n73 = xnode "Read/Write Control"("FPGA VI Reference In"=w965, "error in"=w974, "Value"=w959) -> ("FPGA VI Reference Out"=w966:refnum<k20>, "error out"=w973:errorcluster)
        }
        frame "Digital PWM Out" {
          n74 = Array Subset(array=w1023, index=w1021, length=w1022) -> (w1020:dbl[])
          n75 = Index Array(array=w1020) -> (element #1=w1015:dbl, element #2=w1013:dbl, element #3=w1014:dbl)  [unwired: 3 in]
          n76 = To Single Precision Float(number=w1013) -> (single precision float=w1007:sgl)
          n77 = To Single Precision Float(number=w1014) -> (single precision float=w1006:sgl)
          n78 = In Range and Coerce(upper limit=sgl 100.0, x=w1006, lower limit=sgl 0.0) -> (coerced(x)=w1005:sgl)  [unwired: 1 out]
          n79 = Equal To 0?(x=w1007) -> (x = 0?=w1012:bool)
          n80 = Divide(x=sgl 40000000.0 ("y"), y=w1007) -> (x/y=w1010:sgl)
          n81 = Multiply(x=w1005, y=sgl 0.01 ("x")) -> (x*y=w1008:sgl)
          n82 = case shown="True" w1012 {
            tunnel: [w1044 w1045] -> w1011
            tunnel: w1010 -> [w1044 _]
            tunnel: [w1043 w1045] -> w1009
            tunnel: w1008 -> [w1043 _]
            frame False {
            }
            frame True {
              w1045 = sgl 0.0
            }
          }
          n83 = Greater?(x=w1015, y=0.5) -> (0:w1018:bool)
          n84 = To Unsigned Long Integer(number=w1011) -> (unsigned 32bit integer=w1025:u32)
          n85 = Multiply(x=w1011, y=w1009) -> (x*y=w1017:u32)
          n86 = Subtract(x=w1025, y=w1017) -> (x-y=w1016:u32)
          n87 = Bundle By Name(cluster=T5 {"ACTIVE EDGE"=FALSE, "ACTIVE TICKS"=0, "INACTIVE TICKS"=0} ("Value"), "ACTIVE EDGE"=w1018, "ACTIVE TICKS"=w1017, "INACTIVE TICKS"=w1016) -> (w1000:T5)
          n88 = xnode "Read/Write Control"("FPGA VI Reference In"=w1028, "error in"=w1030, "Value"=w1000) -> ("FPGA VI Reference Out"=w1027:refnum<k20>, "error out"=w1029:errorcluster)
        }
        frame "Digital WSS Out" {
          # "Speed\nData\nPPR\nWD\nSensor"
          n89 = Array Subset(array=w1082, index=w1080, length=w1081) -> (w1079:dbl[])
          n90 = Index Array(array=w1079) -> (element #1=w1062:dbl, element #2=w1061:dbl, element #3=w1060:dbl, element #4=w1059:dbl, element #5=w1058:dbl)  [unwired: 5 in]
          n91 = Absolute Value(x=w1062) -> (abs(x)=w1046:dbl)
          n92 = To Single Precision Float(number=w1059) -> (single precision float=w1053:sgl)
          n93 = To Single Precision Float(number=w1046) -> (single precision float=w1055:sgl)
          n94 = To Single Precision Float(number=w1060) -> (single precision float=w1054:sgl)
          n95 = call "WSS_Data_Conversion.vi"("WD"=w1053, "PPR"=w1054, "Speed"=w1055) -> ("Inactive"=w1051:u32, "Active"=w1052:u32)  [unwired: 7 in]
          n96 = To Unsigned Byte Integer(number=w1061) -> (unsigned 8bit integer=w1056:u8)
          n97 = To Unsigned Byte Integer(number=w1058) -> (unsigned 8bit integer=w1057:u8)
          n98 = Bundle By Name(cluster=T6 {"ACTIVE EDGE"=TRUE, "ACTIVE TICKS"=0, "INACTIVE TICKS"=0, "DATA"=0, "SENSOR TYPE"=0} ("Settings"), "ACTIVE EDGE"=TRUE, "ACTIVE TICKS"=w1052, "INACTIVE TICKS"=w1051, "DATA"=w1056, "SENSOR TYPE"=w1057) -> (w1077:T6)
          n99 = xnode "Read/Write Control"("FPGA VI Reference In"=w1064, "error in"=w1084, "Value"=w1077) -> ("FPGA VI Reference Out"=w1065:refnum<k20>, "error out"=w1083:errorcluster)
        }
        frame "Sine Out" {
          n100 = Array Subset(array=w1124, index=w1122, length=w1123) -> (w1121:dbl[])
          n101 = Index Array(array=w1121) -> (element #1=w1114:dbl, element #2=w1115:dbl, element #3=w1116:dbl)  [unwired: 3 in]
          n102 = Divide(x=w1116, y=sgl 40000000.0) -> (x/y=w1113:dbl)
          n103 = Bundle By Name(cluster=T7 {"AMP"=0.0, "OFFSET"=0.0, "PERIODS/TICKS"=0.0} ("Value"), "AMP"=w1114, "OFFSET"=w1115, "PERIODS/TICKS"=w1113) -> (w1111:T7)
          n104 = xnode "Read/Write Control"("FPGA VI Reference In"=w1120, "error in"=w1126, "Value"=w1111) -> ("FPGA VI Reference Out"=w1119:refnum<k20>, "error out"=w1125:errorcluster)
        }
        frame "Digital Static In Settings" {
          n105 = Array Subset(array=w1166, index=w1164, length=w1165) -> (w1149:dbl[])
          n106 = Index Array(array=w1149) -> (element=w1154:dbl)  [unwired: 1 in]
          n107 = Greater?(x=w1154, y=0.5) -> (0:w1152:bool)
          n108 = Bundle By Name(cluster=cluster{"ACTIVE EDGE":bool} {"ACTIVE EDGE"=FALSE} ("Value"), "ACTIVE EDGE"=w1152) -> (w1145:cluster{"ACTIVE EDGE":bool})
          n109 = xnode "Read/Write Control"("FPGA VI Reference In"=w1147, "error in"=w1150, "Value"=w1145) -> ("FPGA VI Reference Out"=w1144:refnum<k20>, "error out"=w1151:errorcluster)
        }
        frame "Digital Static Out" {
          w1187 = 0.5 ("y")
          n110 = Array Subset(array=w1206, index=w1204, length=w1205) -> (w1203:dbl[])
          n111 = Index Array(array=w1203) -> (element #1=w1188:dbl, element #2=w1186:dbl)  [unwired: 2 in]
          n112 = Greater?(x=w1188, y=w1187) -> (0:w1184:bool)
          n113 = Greater?(x=w1186, y=w1187) -> (0:w1185:bool)
          n114 = Bundle By Name(cluster=cluster{"ACTIVE EDGE":bool, "OUTPUT":bool} {"ACTIVE EDGE"=FALSE, "OUTPUT"=FALSE} ("Value"), "ACTIVE EDGE"=w1184, "OUTPUT"=w1185) -> (w1183:cluster{"ACTIVE EDGE":bool, "OUTPUT":bool})
          n115 = xnode "Read/Write Control"("FPGA VI Reference In"=w1191, "error in"=w1208, "Value"=w1183) -> ("FPGA VI Reference Out"=w1190:refnum<k20>, "error out"=w1207:errorcluster)
        }
        frame "Quad Encoder Settings" {
          w1226 = 0.5 ("y")
          n116 = Array Subset(array=w1252, index=w1250, length=w1251) -> (w1249:dbl[])
          n117 = Index Array(array=w1249) -> (element #1=w1223:dbl, element #2=w1224:dbl, element #3=w1227:dbl, element #4=w1228:dbl, element #5=w1229:dbl)  [unwired: 5 in]
          n118 = Greater?(x=w1227, y=w1226) -> (0:w1225:bool)
          n119 = Greater?(x=w1228, y=w1226) -> (0:w1236:bool)
          n120 = Greater?(x=w1229, y=w1226) -> (0:w1237:bool)
          n121 = Bundle By Name(cluster=T8 {"DIRECTION"=0, "RESET VALUE"=0, "A RESET STATE"=FALSE, "B RESET STATE"=FALSE, "Z RESET STATE"=FALSE} ("Value"), "DIRECTION"=w1223, "RESET VALUE"=w1224, "A RESET STATE"=w1225, "B RESET STATE"=w1236, "Z RESET STATE"=w1237) -> (w1230:T8)
          n122 = xnode "Read/Write Control"("FPGA VI Reference In"=w1234, "error in"=w1254, "Value"=w1230) -> ("FPGA VI Reference Out"=w1232:refnum<k20>, "error out"=w1253:errorcluster)
        }
      }
      n123 = Bundle By Name(cluster=w107, "Quad Encoder Settings"=w50, "Digital WSS Out"=w52, "Digital Static Out"=w56, "Digital Static In Settings"=w55, "Sine Out"=w74, "Digital PWM In Settings"=w79, "Analog PWM In Settings"=w80, "Digital PWM Out"=w83, "U64"=w89, "U32"=w91, "U16"=w93, "U8"=w95, "I64"=w97, "I32"=w99, "I16"=w101, "I8"=w106, "SGL"=w105, "Bool"=w102, "FXP+/-24.5"=w66, "FXP+/-16.5"=w69, "FXP+/-32.8"=w70, "FXP+/-64.32"=w73, "FXP+/-16.7"=w64, "FXP+/-20.5"=w62, "FXP+/-27.5"=w60, "FXP+/-32.16"=w58, "FXP+16.3"=w48, "FXP+18.3"=w46) -> (w87:T1)
    }
  }
  "error out" <- w39
  "Cluster" <- w28
  "Values" <- w27
